vi "GEMM_Top.vi"() -> ()   [LabVIEW 2020]
doc: "This benchmark is designed to demonstrate execution performance improvement when executing FFT and IFFT operations on a GPU."
uses:
  <vilib>/Utility/file.llb/Read Delimited Spreadsheet (DBL).vi
  <vilib>/Analysis/1siggen.llb/Ramp Pattern by Delta.vi
  <vilib>/Ngene/CuLab - GPU Accelerated Toolkit/Toolkit/CuLab.lvlib
  <vilib>/Analysis/NI_AALBase.lvlib
panel:
  in  "CPU Iteration":i32=3
  out "CuLab Mean Performance Gain":dbl[](array[numeric])=[1.0, 32.70718635151803, 2.5525467614410227] format="%#.2g"
  out "Releative Exec Time vs CuLab":cluster{i32[], "all rows":dbl[]}[](graph)=[{[64, 128, 256, 512, 1024, 2048, 4096, 8192], "all rows"=[1.0, 1.0, 1.0, 1.0, 1.0, 1.0, 1.0, 1.0]}, {[64, 128, 256, 512, 1024, 2048, 4096, 8192], "all rows"=[0.2133838298871944, 1.4083191819921286, 3.1841059555062183, 8.844266159971816, 21.725846108107117, 43.56006909698582, 73.31376485796767, 109.40773562172632]}, {[64, 128, 256, 512, 1024, 2048, 4096, 8192], "all rows"=[7.09343425544868, 4.483870959156996, 1.9112582757762941, 1.4608305799968355, 1.356595313756594, 1.4699518137900995, 1.3925360760265713, 1.251896817576111]}]
  in  "CuPy CSV":path=path "D:/Ngene/GitHub/culab_examples/Benchmarks/CuPy/results/GeForce_RTX_2080_Ti/GEMM_CuPy.csv"
  out "Execution Time":cluster{i32[], "all rows":dbl[]}[](graph)=[{[64, 128, 256, 512, 1024, 2048, 4096, 8192], "all rows"=[3.960000049119117e-05, 5.890000011277152e-05, 0.00015100000018719584, 0.00042380000013508834, 0.0013828000001012697, 0.005499500000041735, 0.02617389999977604, 0.1437802999998894]}, {[64, 128, 256, 512, 1024, 2048, 4096, 8192], "all rows"=[8.449999768345151e-06, 8.294999997815466e-05, 0.00048079999987749034, 0.0037481999997908133, 0.03004250000049069, 0.2395586000006915, 1.9189071499995407, 15.730677050000395]}, {[64, 128, 256, 512, 1024, 2048, 4096, 8192], "all rows"=[0.0002809, 0.0002641, 0.0002886, 0.0006191, 0.0018759000000000002, 0.008084000000000001, 0.036448100000000004, 0.17999810000000002]}]
  out "GPU Model":string="NVIDIA GeForce RTX 2080 Ti"
  out "CPU Model":string="Intel(R) Core(TM) i7-8700K"
  in  "GPU Iteration":i32=50
  in  "Size Stop(2^n)":i32=13
  in  "Size Start(2^n)":i32=6
  out "Dims H,W":i32[](array[numeric])=[64, 128, 256, 512, 1024, 2048, 4096, 8192] format="%.2p"
  # "GEMM Benchmark"
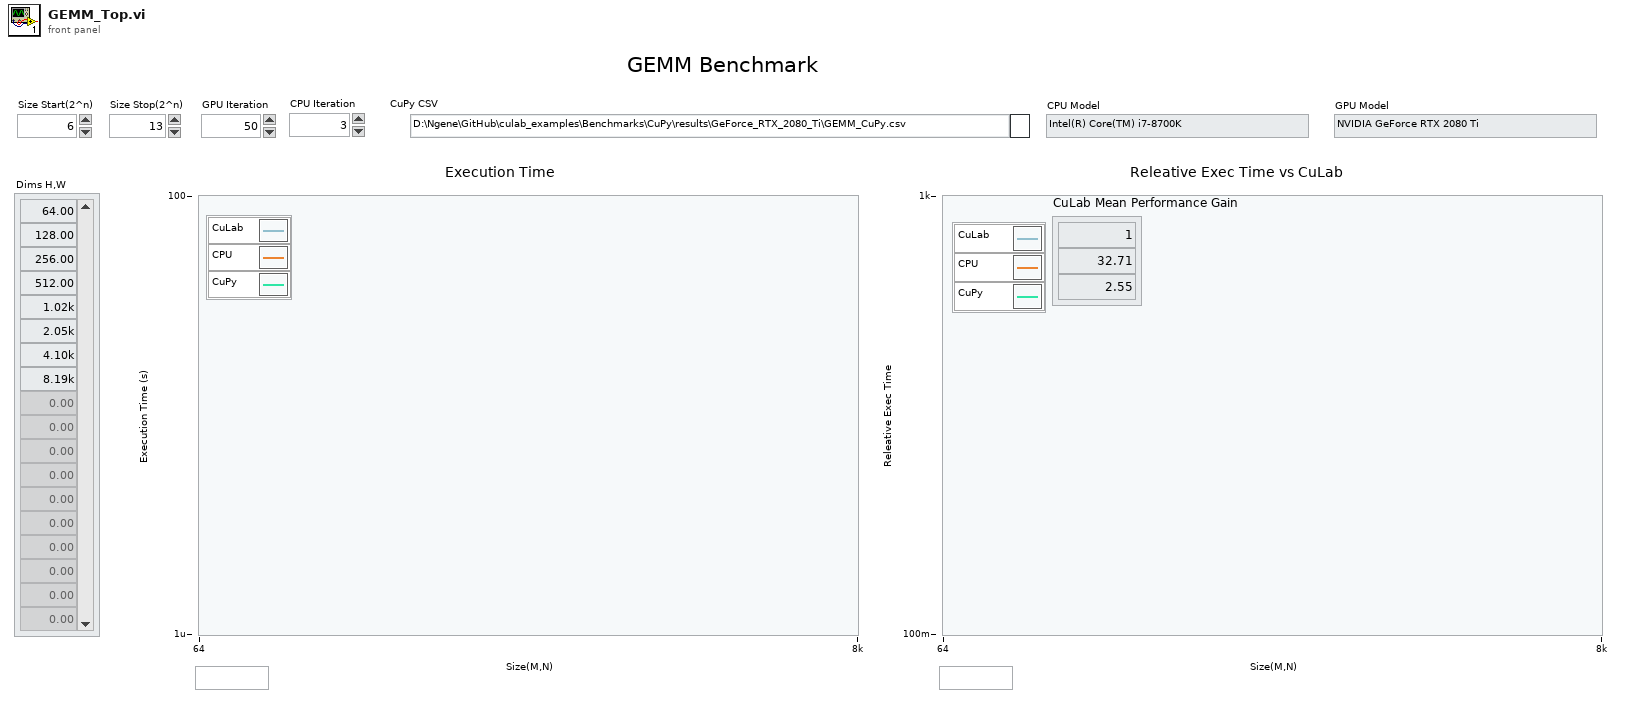
[diagram p1: front panel]
types:
  T1 = typedef "CuLab.lvlib/Properties.ctl" = cluster{"Device ID":i32, "Name":string}
  T2 = typedef "imagedata.ctl" = cluster{"image type":i32, "image depth":i32, "image":u8[], "mask":u8[], "colors":u32[], "Rectangle":cluster{"left":i16, "top":i16, "right":i16, "bottom":i16}}
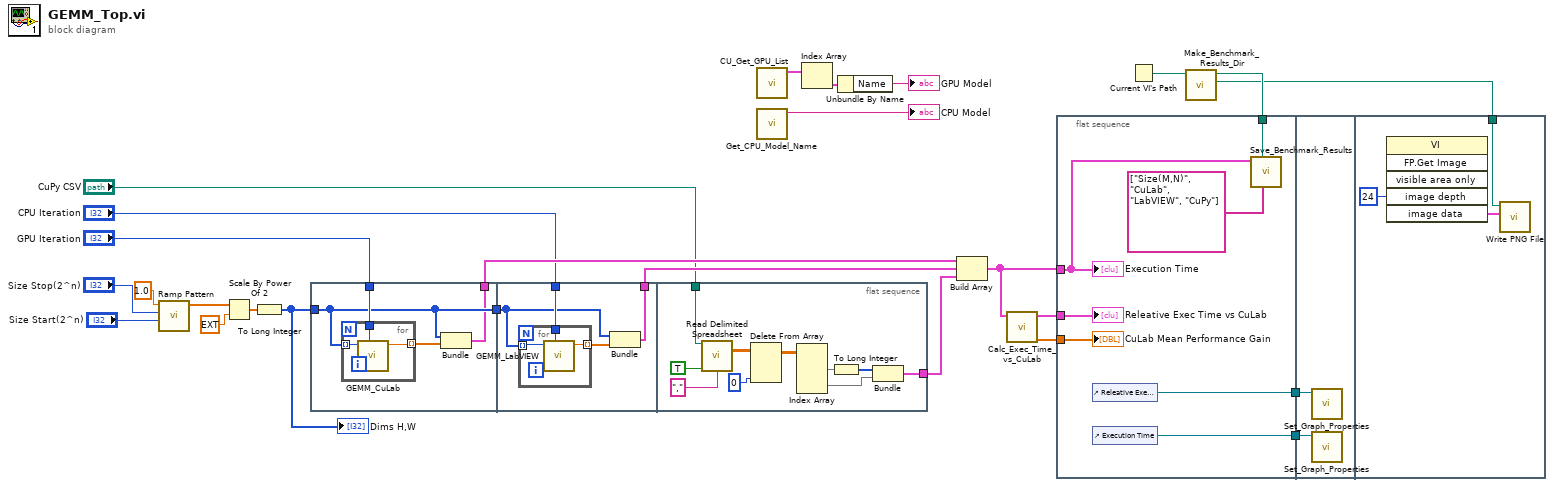
[diagram p0: block diagram]
diagram:
  n1 = call-poly <vilib>:"Ramp Pattern.vi"("start"="Size Start(2^n)", "end"="Size Stop(2^n)", "delta"=1.0) -> ("Ramp Pattern"=w11:dbl[])  [unwired: 6 in, 2 out]
  n2 = Scale By Power Of 2(n=w11, x=ext 1.0) -> (x*2^n=w13:ext[])
  n3 = To Long Integer(number=w13) -> (32bit integer=w10:i32[])
  "Dims H,W" <- w10
  n4 = flat-sequence {
    tunnel: [w27] -> w22
    tunnel: [w28] -> w23
    tunnel: w10 -> [w28]
    tunnel: "GPU Iteration" -> [w30]
    tunnel: w23 -> [w35]
    tunnel: "CPU Iteration" -> [w37]
    tunnel: [w34] -> w21
    tunnel: "CuPy CSV" -> [w50]
    tunnel: [w42] -> w19
    frame #0 {
      n5 = for {
        tunnel: w30 -> [w31]
        tunnel: w28 -> [w32] mode=indexing
        tunnel: [w33] -> w29 mode=indexing
        n6 = call "GEMM_CuLab.vi"("Iteration"=w31, "Size"=w32) -> ("Result(s)"=w33:dbl)  [unwired: 9 in]
      }
      n7 = Bundle(w28, w29) -> (w27:cluster{i32[], dbl[]})  [unwired: 1 in]
    }
    frame #1 {
      n8 = for {
        tunnel: w35 -> [w40] mode=indexing
        tunnel: w37 -> [w38]
        tunnel: [w39] -> w36 mode=indexing
        n9 = call "GEMM_LabVIEW.vi"("Iteration"=w38, "Size"=w40) -> ("Result(s)"=w39:dbl)  [unwired: 9 in]
      }
      n10 = Bundle(w35, w36) -> (w34:cluster{i32[], dbl[]})  [unwired: 1 in]
    }
    frame #2 {
      n11 = call-poly <vilib>:"Read Delimited Spreadsheet.vi"("file path (dialog if empty)"=w50, "transpose? (F)"=TRUE, "delimiter (\\t)"="," ("delimiter (\\t)")) -> ("all rows"=w48:dbl[][])  [unwired: 7 in, 5 out]
      n12 = Delete From Array(array=w48, index (col)=0 ("disabled index (col)")) -> (array with subset deleted=w46:dbl[][])  [unwired: 2 in, 1 out]
      n13 = Index Array(array=w46) -> (element #1=w45:dbl[], element #2=w43:dbl[])  [unwired: 4 in]
      n14 = To Long Integer(number=w45) -> (32bit integer=w44:i32[])
      n15 = Bundle(w44, "all rows"=w43) -> (w42:cluster{i32[], "all rows":dbl[]})  [unwired: 1 in]
    }
  }
  n16 = call <vilib>:"CU_Get_GPU_List.vi"() -> ("Devices"=w25:T1[])  [unwired: 10 in, 1 out]
  n17 = call "Get_CPU_Model_Name.vi"() -> ("CPU Model"=→"CPU Model":string)  [unwired: 11 in]
  n18 = Index Array(array=w25) -> (element=w24:T1)  [unwired: 1 in]
  n19 = Unbundle By Name(w24) -> ("Name"=→"GPU Model":string)
  n20 = Build Array(w22, w21, w19) -> (w17:cluster{i32[], "all rows":dbl[]}[])
  n21 = call "Calc_Exec_Time_vs_CuLab.vi"("Exec Times"=w17) -> ("Mean Gain"=w1:dbl[], "CuLab Gain"=w18:cluster{"Array":i32[], "all rows":dbl[]}[])  [unwired: 9 in]
  n22 = flat-sequence {
    tunnel: w18 -> [w57]
    tunnel: w1 -> [w56]
    tunnel: w17 -> [w53]
    tunnel: w5 -> [w54]
    tunnel: [w52] -> w3
    tunnel: [w51] -> w2
    tunnel: w3 -> [w59]
    tunnel: w2 -> [w58]
    tunnel: w4 -> [w60]
    frame #0 {
      n23 = control-ref of="Releative Exec Time vs CuLab"() -> (w52:refnum<vi>)
      n24 = control-ref of="Execution Time"() -> (w51:refnum<vi>)
      n25 = call "Save_Benchmark_Results.vi"("Header"=string[] ["Size(M,N)", "CuLab", "LabVIEW", "CuPy"], "file path (dialog if empty)"=w54, "Execution Time"=w53) -> ()  [unwired: 9 in]
      "Execution Time" <- w53
      "CuLab Mean Performance Gain" <- w56
      "Releative Exec Time vs CuLab" <- w57
    }
    frame #1 {
      n26 = call "Set_Graph_Properties.vi"("Graph"=w59) -> ()  [unwired: 11 in]
      n27 = call "Set_Graph_Properties.vi"("Graph"=w58) -> ()  [unwired: 11 in]
    }
    frame #2 {
      n28 = invoke class="VI" method="FP.Get Image"("image depth"=24 ("Image Depth")) -> ("image data"=w62:T2)  [unwired: 5 in, 5 out]
      n29 = call <vilib>:"Write PNG File.vi"("image data"=w62, "path to PNG file"=w60) -> ()  [unwired: 8 in, 2 out]
    }
  }
  n30 = Current VI's Path() -> (path=w6:path)
  n31 = call "Make_Benchmark_Results_Dir.vi"("Caller Path"=w6) -> ("Caller FP Image Path"=w4:path, "CSV_File"=w5:path)  [unwired: 9 in]
